vi "Create Error.vi"(5 "Local Context (None)":string, 7 "Call Chain (F)":bool, 9 "MultiErrors in":refnum<class "MultiErrors.lvclass">, 10 "Message":string, 11 "Code":i32=1) -> (1 "MultiErrors out":refnum<class "MultiErrors.lvclass">)   [LabVIEW 2020, in "VolatusErrorUtilities.lvlib" / "MultiErrors.lvclass"]
uses:
  MultiErrors.lvclass
  MultiError.ctl
  MultiErrors.lvclass/MultiErrors.ctl
  VolatusErrorUtilities.lvlib
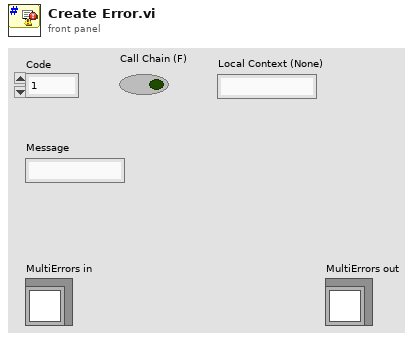
[diagram p1: front panel]
types:
  T1 = typedef "VolatusErrorUtilities.lvlib/MultiError.ctl" = cluster{"Context":string[], "Message":string, "Code":i32, "Call Chain":string[]}
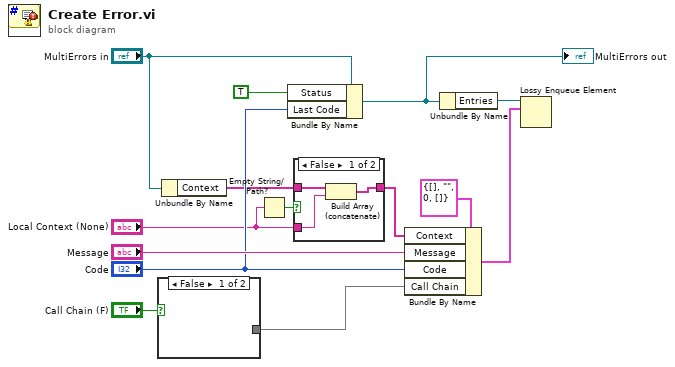
[diagram p0: block diagram]
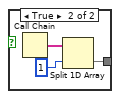
[diagram p3: hidden frame]
diagram:
  n1 = case shown="False" "Call Chain (F)" {
    tunnel: [_ w15] -> w11
    frame False {
    }
    frame True {
      n2 = Call Chain() -> (call chain=w17:string[])
      n3 = Split 1D Array(array=w17, index=1) -> (second subarray=w15:string[])  [unwired: 1 out]
    }
  }
  n4 = Unbundle By Name("MultiErrors in") -> ("Context"=w2:string[])
  n5 = Empty String/Path?(string/path="Local Context (None)") -> (empty?=w3:bool)
  n6 = Bundle By Name(cluster="MultiErrors in", "Status"=TRUE, "Last Code"="Code") -> (w7:refnum<class "MultiErrors.lvclass">)
  "MultiErrors out" <- w7
  n7 = case shown="False" w3 {
    tunnel: "Local Context (None)" -> [w19 _]
    tunnel: w2 -> [w20 w21]
    tunnel: [w18 w21] -> w1
    frame False {
      n8 = Build Array (concatenate)(w20, w19) -> (w18:string[])
    }
    frame True {
    }
  }
  n9 = Bundle By Name(cluster=T1 {"Context"=[], "Message"="", "Code"=0, "Call Chain"=[]} ("MultiError Entry"), "Context"=w1, "Message"="Message", "Code"="Code", "Call Chain"=w11) -> (w9:T1)
  n10 = Unbundle By Name(w7) -> ("Entries"=w10:refnum<queue>)
  n11 = Lossy Enqueue Element(queue=w10, element=w9) -> ()  [unwired: 1 in, 4 out]
